vi "Microscope.Initialized.vi"(8 "error in (no error)":errorcluster, 10 "Initialized":T1, 11 "Microscope":refnum<class "Microscope.lvclass">) -> (0 "error out":errorcluster, 3 "Microscope out":refnum<class "Microscope.lvclass">)   [LabVIEW 2013, in "Microscope.lvclass"]
doc: "---------------------------------------------------------------\nJKI State Machine Objects™\nhttp://jki.net/state-machine-objects/\nCopyright (C) 2005-2015, JKI <info@jki.net>\nALL RIGHTS RESERVEDJKI State Machine Objects (SMO) 1.0.0.4\nJKI - JKI\nCopyright (c) 2015, JKI"
uses:
  Microscope.lvclass
  Typedefs/PublicEvents--Microscope.Initialized.ctl
panel:
  # "For instructions on how to use the JKI State Machine Objects, examples and video tutorials, visit:\nhttp://jki.net/state-machine-objects/\n\nJKI State Machine Objects™\nhttp://jki.net/state-machine-objects/\nCopyright (C) 2005-2015, JKI <info@jki.net>\nALL RIGHTS RESERVED"
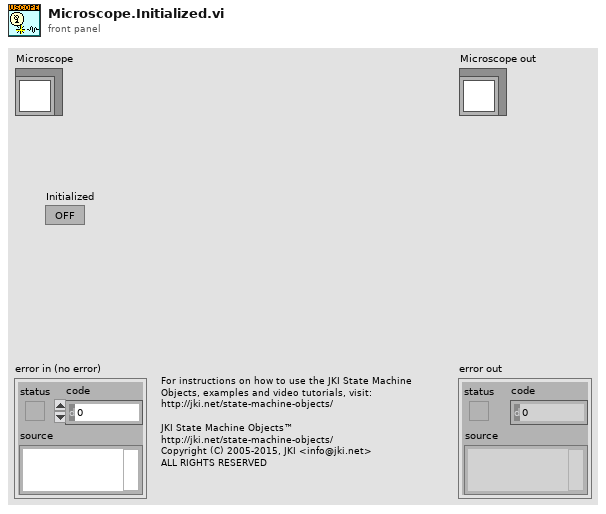
[diagram p1: front panel]
types:
  T1 = typedef "Microscope.lvclass/PublicEvents--Microscope.Initialized.ctl" = bool
  T2 = typedef "Microscope.lvclass/PublicEvents--Cluster.ctl" = cluster{"Value Changed":refnum<user-event>, "Initialized":refnum<user-event>}
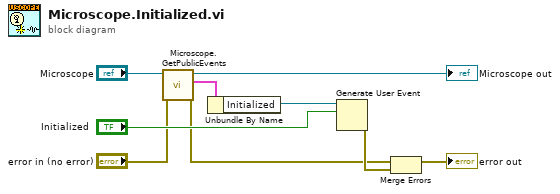
[diagram p0: block diagram]
diagram:
  n1 = call "Microscope.GetPublicEvents.vi"("error in (no error)"="error in (no error)", "Microscope"="Microscope") -> ("error out"=w1:errorcluster, "Microscope Public Events"=w6:T2, "Microscope out"=→"Microscope out":refnum<class "Microscope.lvclass">)  [unwired: 7 in]
  n2 = Unbundle By Name(w6) -> ("Initialized"=w5:refnum<user-event>)
  n3 = Generate User Event(user event=w5, event data cluster="Initialized") -> (error out=w4:errorcluster)  [unwired: 2 in, 1 out]
  n4 = Merge Errors(w1, w4) -> (→"error out":errorcluster)
